vi "[ce] CalcExpress.vi"(4 "directives":T1={"enaNamedConst"=TRUE}, 5 "VC Handle":T4=-1, 6 "error in":errorcluster, 7 "params":T5={"autoVar"=TRUE, "enCpx"=TRUE}, 8 "repeat (1)":i32=1, 9 "expression":string) -> (0 "error out":errorcluster, 1 "value type":T3=enum."DBL Number", 2 "string value":string, 3 "numeric value":dbl)   [LabVIEW 2021]
doc: "This VI evaluates CalcExpress expressions and sequential scripts. To process non-sequential scripts that contain loops and conditional branching, use <b>CSE VIs</b>. Refer to the VI help for more details.\n\n<b>VC Handle</b> specifies the handle of a variable context. CalcExpress accesses variables using this handle. Pass a valid handle to this terminal if the expression uses variables; otherwise, you can leave this input unwired.\n\n<b>expression</b> specifies the CalcExpress expression or sequential script to be executed.\n\n<b>repeat</b> control specifies the number of times an expression is evaluated. The default value is 1.\n\n<b>params</b> cluster specifies optional parameters influencing evaluation:\n <b>autoVar</b> : if it is TRUE (default) and a non-existent variable appears as the left-hand operand in the assignment operator, CalcExpress implicitly creates the variable. If it is FALSE, all variables in the expression must be explicitly created either before or during evaluation.\n <b>enCpx</b> : enables (TRUE, default) or disables (FALSE) the ability to perform operations on operands of data types other than <b>DBL Number</b>.\n\n<b>numeric value</b> returns the numeric value (<b>DBL Number</b>) of the expression.\n\n<b>string value</b> returns the non-numeric value of the expression. The value is represented in the LabVIEW Flattened-To-String format unless the data type of the expression is <b>String</b>.\n\n<b>value type</b> indicates the data type of the expression value.\n\n::: CalcExpress Toolkit :::\nCopyright (c) 2000-2026 Konstantin Shifershteyn. All rights reserved."
uses:
  cetypes.llb/CalcExpress Execution Options.ctl
  cetypes.llb/VarMan Variable Context Handle.ctl
  cetypes.llb/CalcExpress Data Type.ctl
  cetypes.llb/CalcExpress Instance RefNum.ctl
  cetypes.llb/CalcExpress Parsing Directives.ctl
  cersrc/celveng32.dll
panel:
  in  "CE InstanceRef Templ.":T2
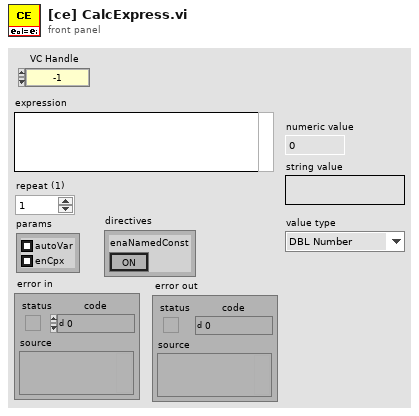
[diagram p1: front panel]
types:
  T1 = typedef "CalcExpress Parsing Directives.ctl" = cluster{"enaNamedConst":bool}
  T2 = typedef "CalcExpress Instance RefNum.ctl" = refnum<k1>
  T3 = typedef "CalcExpress Data Type.ctl" = enum32{"String", "DBL Number", "identifier", "1D Array of DBL", "2D Array of DBL", "CDB Number", "1D Array of CDB", "2D Array of CDB", "1D Array of String", "2D Array of String", "Unknown data type"}
  T4 = typedef "VarMan Variable Context Handle.ctl" = i32
  T5 = typedef "CalcExpress Execution Options.ctl" = cluster{"autoVar":bool, "enCpx":bool}
  T6 = enum32{"String", "DBL Number", "identifier", "1D Array of DBL", "2D Array of DBL", "CDB Number", "1D Array of CDB", "2D Array of CDB", "1D Array of String", "2D Array of String", "Unknown data type"}
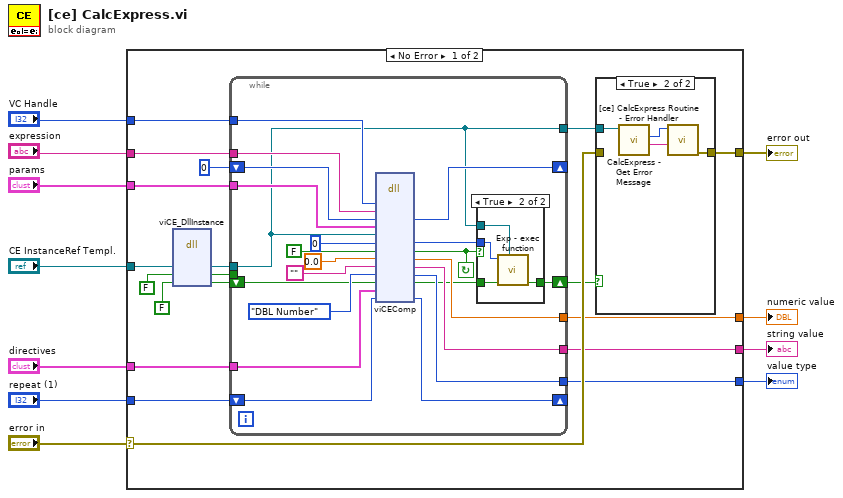
[diagram p0: block diagram]
diagram:
  n1 = case shown="No Error" "error in" {
    selector: "error in" -> [w17 w63]
    tunnel: "CE InstanceRef Templ." -> [w27 _]
    tunnel: "repeat (1)" -> [w25 _]
    tunnel: "VC Handle" -> [w23 _]
    tunnel: "expression" -> [w22 _]
    tunnel: "params" -> [w21 _]
    tunnel: [w20 w63] -> w6
    tunnel: [w16 _] -> w4
    tunnel: [w15 _] -> w3
    tunnel: [w14 _] -> w2
    tunnel: "directives" -> [w12 _]
    frame No Error {
      n2 = dll-call lib="C:/LV Projects/CalcExpress 40 LV2021/vi.lib/addons/CalcExpress/cersrc/celveng*.dll" fn="viCE_DllInstance"("iRef"=w27, "newInst"=FALSE, "err_f"=FALSE) -> ("iRef"=w30:T2, "newInst"=w19:bool, "err_f"=w29:bool)  [unwired: 6 in, 2 out]
      n3 = while {
        tunnel: [w33] -> w26
        shift-left: w25 -> [w34]
        shift-right: [w35] -> _
        tunnel: [w39] -> w15
        tunnel: [w38] -> w16
        tunnel: [w40] -> w14
        tunnel: w30 -> [w33]
        tunnel: w22 -> [w50]
        tunnel: w23 -> [w51]
        tunnel: w21 -> [w48]
        shift-left: 0 -> [w49]
        shift-right: [w43] -> _
        shift-left: w29 -> [w37]
        shift-right: [w52] -> w13
        tunnel: w19 -> [_]
        tunnel: w12 -> [w31]
        stop <- w41 continue-if-true
        n4 = dll-call lib="C:/LV Projects/CalcExpress 40 LV2021/vi.lib/addons/CalcExpress/cersrc/celveng*.dll" fn="viCEComp"("vch"=w51, "script"=w50, "idx"=w49, "cPar"=w48, "iRef"=w33, "opdNum"=0, "NE"=FALSE, "num"=0.0, "str"="" ("Empty String Constant"), "type"=T6."DBL Number" ("data type"), "erf"=w37, "dirs"=w31, "rept"=w34) -> ("idx"=w43:i32, "opdNum"=w42:i32, "NE"=w41:bool, "num"=w40:dbl, "str"=w39:string, "type"=w38:T6, "erf"=w36:bool, "rept"=w35:i32)  [unwired: 9 in, 2 out]
        n5 = case shown="True" w41 {
          tunnel: [w53 w57] -> w52
          tunnel: w36 -> [w53 w56]
          tunnel: w42 -> [_ w55]
          tunnel: w33 -> [_ w54]
          frame False {
          }
          frame True {
            n6 = call "Exp - exec function.vi"("CE InstanceRef"=w54, "error in"=w56, "ParNum"=w55) -> ("error out"=w57:bool)  [unwired: 6 in]
          }
        }
      }
      n7 = case shown="True" w13 {
        tunnel: w26 -> [_ w62]
        tunnel: [w58 w59] -> w20
        tunnel: w17 -> [w58 _]
        frame False {
        }
        frame True {
          n8 = call "CalcExpress - Get Error Message.vi"("CE InstanceRef"=w62) -> ("error description"=w61:string, "error code"=w60:i32)  [unwired: 5 in, 2 out]
          n9 = call "[ce] CalcExpress Routine - Error Handler.vi"("error msg"=w61, "error code"=w60) -> ("error out"=w59:errorcluster)  [unwired: 7 in]
        }
      }
    }
    frame Error {
    }
  }
  "error out" <- w6
  "numeric value" <- w2
  "string value" <- w3
  "value type" <- w4
